vi "detect controller.vi"() -> (0 "error out":errorcluster, 2 "passed?":bool)   [LabVIEW 2014, in "tests.lvlib"]
uses:
  tests.lvlib
  classes/SysCfg Device/SysCfg Device.lvclass
  classes/Controller/Controller.lvclass
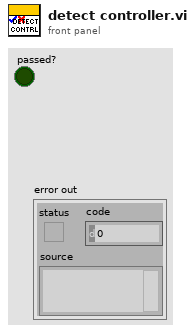
[diagram p1: front panel]
types:
  T1 = typedef "SMI.lvlib/Device.lvclass/login credentials.ctl" = cluster{"device class":string, "hostname":string, "IP address":string, "username":string, "password":string}
  T2 = typedef "SMI.lvlib/Controller.lvclass/controller information.ctl" = cluster{"system session":refnum<data-value>, "system hardware ref":refnum<data-value>, "vendor name":string, "product name":string, "product ID":u16, "serial number":string, "device information":T3, "primary network adapter":T4, "secondary network adapters":T4[]}
  T3 = typedef "SMI.lvlib/Controller.lvclass/device information.ctl" = cluster{"resource":string, "device class":string, "system start time":timestamp, "current time":timestamp, "time zone":string, "firmware revision":string, "image title":string, "image version":string, "system status":string}
  T4 = typedef "SMI.lvlib/Controller.lvclass/network adapter settings.ctl" = cluster{"IP address":string, "MAC address":string, "IP address request mode":u32, "subnet mask":string, "gateway":string, "DNS server":string, "adapter mode":u32, "adapter type":u32}
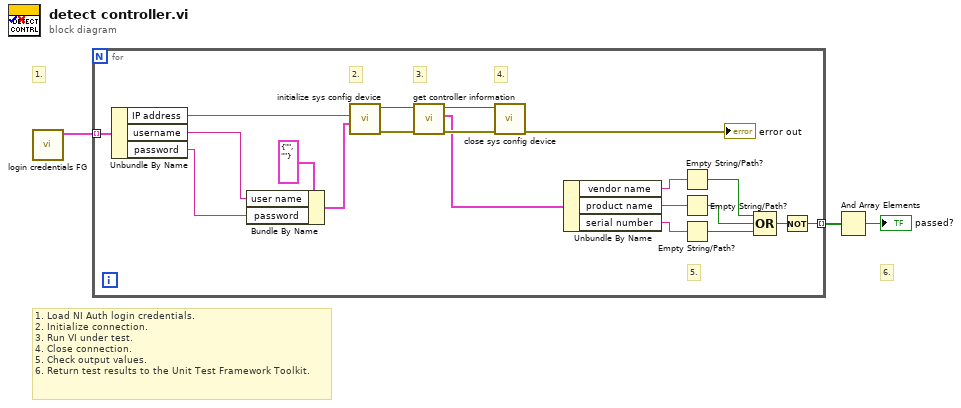
[diagram p0: block diagram]
diagram:
  # "1."
  # "6."
  # "1. Load NI Auth login credentials.\n2. Initialize connection.\n3. Run VI under test.\n4. Close connection.\n5. Check output values.\n6. Return test results to the Unit Test Framework Toolkit."
  n1 = call "login credentials FG.vi"() -> ("login credentials"=w1:T1[])  [unwired: 10 in, 1 out]
  n2 = for {
    tunnel: [w10] -> w2 mode=indexing
    tunnel: w1 -> [w8] mode=indexing
    # "4."
    # "2."
    # "3."
    # "5."
    n3 = Unbundle By Name(w8) -> ("IP address"=w7:string, "username"=w5:string, "password"=w6:string)
    n4 = Bundle By Name(cluster=cluster{"user name":string, "password":string} {"user name"="", "password"=""} ("login"), "user name"=w5, "password"=w6) -> (w21:cluster{"user name":string, "password":string})
    n5 = call "initialize sys config device.vi"("login"=w21, "IP address (localhost)"=w7) -> ("error out"=w23:errorcluster, "controller out"=w20:refnum<class "Controller.lvclass">)  [unwired: 8 in]
    n6 = call "get controller information.vi"("error in"=w23, "controller in"=w20) -> ("error out"=w22:errorcluster, "controller information"=w18:T2, "controller out"=w19:refnum<class "Controller.lvclass">)  [unwired: 7 in]
    n7 = call "close sys config device.vi"("error in"=w22, "controller in"=w19) -> ("error out"=→"error out":errorcluster)  [unwired: 8 in, 1 out]
    n8 = Unbundle By Name(w18) -> ("vendor name"=w16:string, "product name"=w15:string, "serial number"=w17:string)
    n9 = Empty String/Path?(string/path=w16) -> (empty?=w14:bool)
    n10 = Empty String/Path?(string/path=w15) -> (empty?=w13:bool)
    n11 = Empty String/Path?(string/path=w17) -> (empty?=w12:bool)
    n12 = Compound Arithmetic op=OR(w14, w13, w12) -> (w11:bool)
    n13 = Not(x=w11) -> (.not. x?=w10:bool)
  }
  n14 = And Array Elements(Boolean array=w2) -> (logical AND=→"passed?":bool)
